vi "[ce] CalcExpress - Close Instance.vi"(6 "error in":errorcluster, 9 "CE InstanceRef":T1) -> (0 "error out":errorcluster, 1 "destroyed":bool, 3 "dup CE InstanceRef":T1)   [LabVIEW 2021]
doc: "This VI destroys a dynamic CalcExpress instance context or reinitializes a static instance context. Refer to the VI help for more details.\n\n::: CalcExpress Toolkit :::\nCopyright (c) 2000-2026 Konstantin Shifershteyn. All rights reserved."
uses:
  cetypes.llb/CalcExpress Instance RefNum.ctl
  cersrc/celveng32.dll
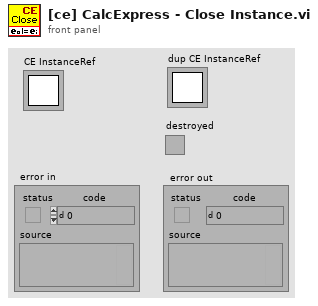
[diagram p1: front panel]
types:
  T1 = typedef "CalcExpress Instance RefNum.ctl" = refnum<k1>
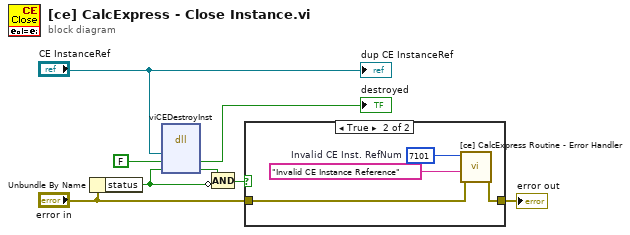
[diagram p0: block diagram]
diagram:
  n1 = Unbundle By Name("error in") -> ("status"=w4:bool)
  n2 = dll-call lib="C:/LV Projects/CalcExpress 40 LV2021/vi.lib/addons/CalcExpress/cersrc/celveng*.dll" fn="viCEDestroyInst"("iRef"="CE InstanceRef", "fDestroyed"=FALSE, "erf"=w4) -> ("fDestroyed"=→"destroyed":bool, "erf"=w5:bool)  [unwired: 5 in, 2 out]
  n3 = Compound Arithmetic op=AND(w5, invert w4) -> (w7:bool)
  n4 = case shown="True" w7 {
    tunnel: "error in" -> [w9 w11]
    tunnel: [w9 w13] -> w6
    frame False {
    }
    frame True {
      w10 = 7101  # Invalid CE Inst. RefNum
      n5 = call "[ce] CalcExpress Routine - Error Handler.vi"("error in"=w11, "error msg"="Invalid CE Instance Reference" ("error description"), "error code"=w10) -> ("error out"=w13:errorcluster)  [unwired: 6 in]
    }
  }
  "error out" <- w6
  "dup CE InstanceRef" <- "CE InstanceRef"
